vi "Enable Monitoring All Labels on Channel.vi"(8 "error in":errorcluster, 10 "channel number":u8, 11 "board handle":u8) -> (0 "error out":errorcluster, 2 "channel number out":u8, 3 "board handle out":u8)   [LabVIEW 2020, in "AIM ARINC 429 Hardware API.lvlib"]
uses:
  AIM ARINC 429 Hardware API.lvlib
  <instrlib>/AIM GmbH/_ARINC-429/subvi/Error Converter (ErrCode or Status).vi
  <instrlib>/AIM GmbH/_ARINC-429/subvi/Get Library Path.vi
  <instrlib>/AIM GmbH/_ARINC-429/VIs/Library/Api429Lib Error Desc Get.vi
  <instrlib>/AIM GmbH/_ARINC-429/subvi/Get Error Number Offset.vi
  <vilib>/Utility/error.llb/Error Cluster From Error Code.vi
  <instrlib>/AIM GmbH/_ARINC-429/AIM429LV.lvlib
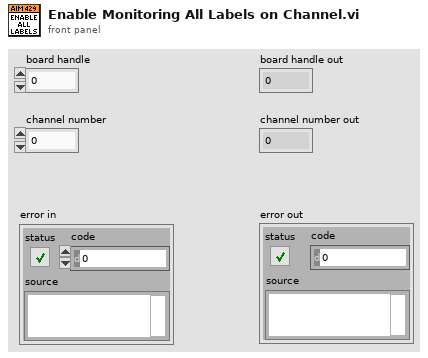
[diagram p1: front panel]
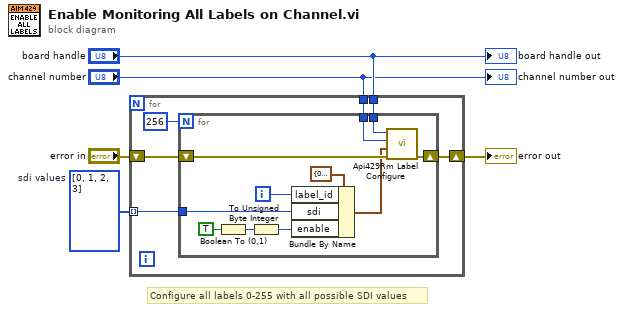
[diagram p0: block diagram]
diagram:
  w1 = u8[] [0, 1, 2, 3]  # sdi values
  # "Configure all labels 0-255 with all possible SDI values"
  n1 = for {
    tunnel: "board handle" -> [w11]
    tunnel: "channel number" -> [w10]
    shift-right: [w8] -> w2
    shift-left: "error in" -> [w9]
    tunnel: w1 -> [w6] mode=indexing
    n2 = for {
      N: 256 -> [_]
      tunnel: w11 -> [w22]
      tunnel: w10 -> [w21]
      shift-right: [w19] -> w8
      shift-left: w9 -> [w20]
      tunnel: w6 -> [w12]
      i -> [w16]
      n3 = Boolean To (0,1)(Boolean=TRUE) -> (0, 1=w14:i16)
      n4 = To Unsigned Byte Integer(number=w14) -> (unsigned 8bit integer=w13:u8)
      n5 = Bundle By Name(cluster=cluster{"label_id":u32, "sdi":u32, "enable":u8} {"label_id"=0, "sdi"=0, "enable"=0} ("label_config"), "label_id"=w16, "sdi"=w12, "enable"=w13) -> (w17:cluster{"label_id":u32, "sdi":u32, "enable":u8})
      n6 = call <instrlib>:"Api429Rm Label Configure.vi"("error in (no error)"=w20, "label_config"=w17, "b_Chn"=w21, "board_handle"=w22) -> ("error out"=w19:errorcluster)  [unwired: 7 in]
    }
  }
  "error out" <- w2
  "board handle out" <- "board handle"
  "channel number out" <- "channel number"
